vi "CARRITO.vi"() -> ()   [LabVIEW 2021]
uses:
  <vilib>/Instr/_visa.llb/VISA Configure Serial Port (Instr).vi
  <vilib>/Utility/inputDevices.llb/keyboardAcquire.vi
  <vilib>/Utility/inputDevices.llb/closeKeyboard.vi
panel:
  out "servo":dbl(knob) scale=-90.0..90.0
  out "Numeric":dbl
  out "VELOCIDAD":dbl(knob) scale=0.0..100.0
  out "keys pressed":T1(array[ring])
  in  "VISA resource name":refnum<visa-resource-name>
  in  "stop":bool
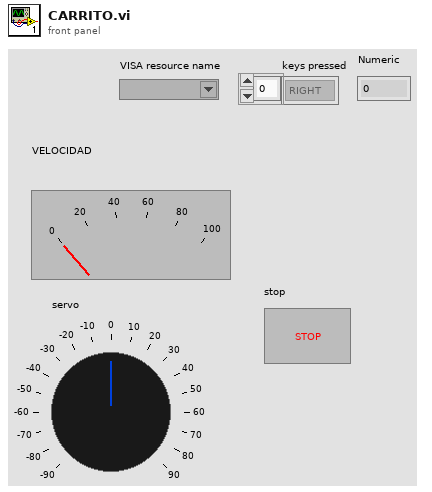
[diagram p1: front panel]
types:
  T1 = enum16{"0", "1", "2", "3", "4", "5", "6", "7", "8", "9", "A", "B", "C", "D", "E", "F", "G", "H", "I", "J", "K", "L", "M", "N", "O", "P", "Q", "R", "S", "T", "U", "V", "W", "X", "Y", "Z", "F1", "F2", "F3", "F4", "F5", "F6", "F7", "F8", "F9", "F10", "F11", "F12", "F13", "F14", "F15", "ADD", "BACK", "BACKSLASH", "CAPITAL", "COMMA", "DECIMAL", "DELETE", "DIVIDE", "DOWN", "END", "EQUALS", "ESCAPE", "GRAVE (`)", "HOME", "INSERT", "LBRACKET", "LCONTROL", "LEFT", "L ALT", "LSHIFT", "LWIN", "MINUS", "MULTIPLY", "NEXT", "NUMLOCK", "NUMPAD_0", "NUMPAD_1", "NUMPAD_2", "NUMPAD_3", "NUMPAD_4", "NUMPAD_5", "NUMPAD_6", "NUMPAD_7", "NUMPAD_8", "NUMPAD_9", "PAUSE", "PERIOD", "PRIOR (PG UP)", "RBRACKET", "RCONTROL", "RETURN", "RIGHT", "R ALT", "RSHIFT", "RWIN", "SCROLL", "SEMICOLON", "SLASH", "SPACE", "SUBTRACT", "TAB", "UP", "ENTER (num pad)", "' (quote)"}[]
  T2 = enum16{"0", "1", "2", "3", "4", "5", "6", "7", "8", "9", "A", "B", "C", "D", "E", "F", "G", "H", "I", "J", "K", "L", "M", "N", "O", "P", "Q", "R", "S", "T", "U", "V", "W", "X", "Y", "Z", "F1", "F2", "F3", "F4", "F5", "F6", "F7", "F8", "F9", "F10", "F11", "F12", "F13", "F14", "F15", "ADD", "BACK", "BACKSLASH", "CAPITAL", "COMMA", "DECIMAL", "DELETE", "DIVIDE", "DOWN", "END", "EQUALS", "ESCAPE", "GRAVE (`)", "HOME", "INSERT", "LBRACKET", "LCONTROL", "LEFT", "L ALT", "LSHIFT", "LWIN", "MINUS", "MULTIPLY", "NEXT", "NUMLOCK", "NUMPAD_0", "NUMPAD_1", "NUMPAD_2", "NUMPAD_3", "NUMPAD_4", "NUMPAD_5", "NUMPAD_6", "NUMPAD_7", "NUMPAD_8", "NUMPAD_9", "PAUSE", "PERIOD", "PRIOR (PG UP)", "RBRACKET", "RCONTROL", "RETURN", "RIGHT", "R ALT", "RSHIFT", "RWIN", "SCROLL", "SEMICOLON", "SLASH", "SPACE", "SUBTRACT", "TAB", "UP", "ENTER (num pad)", "' (quote)"}
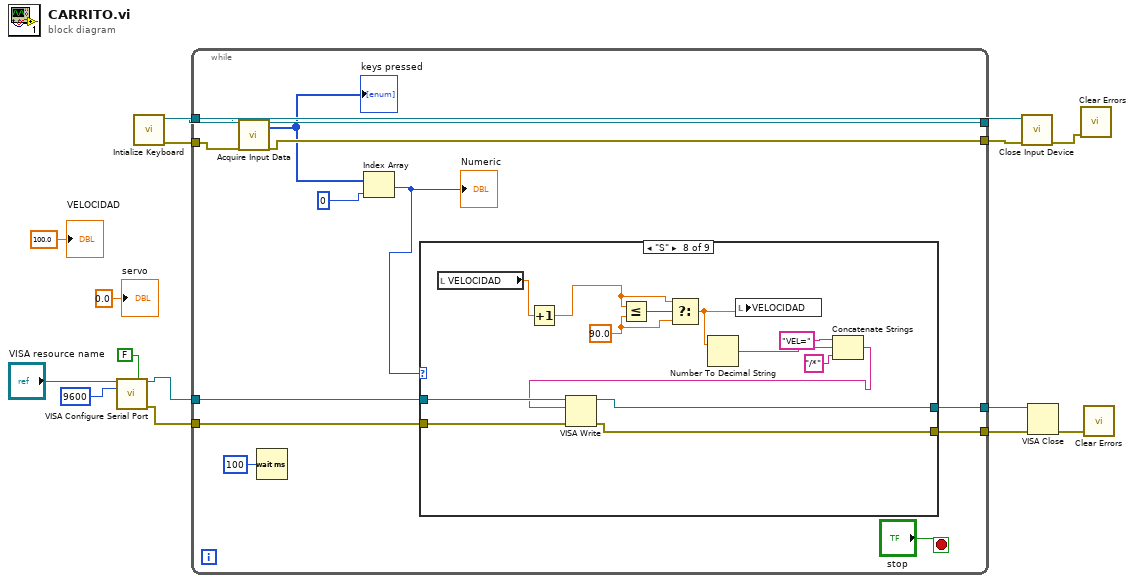
[diagram p0: block diagram]
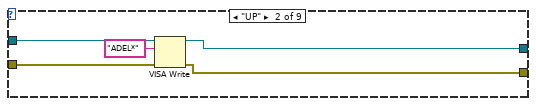
[diagram p3: hidden frame]
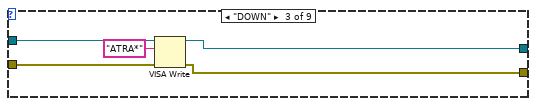
[diagram p4: hidden frame]
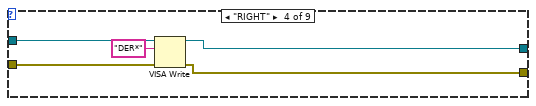
[diagram p5: hidden frame]
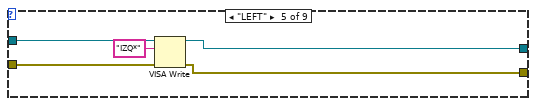
[diagram p6: hidden frame]
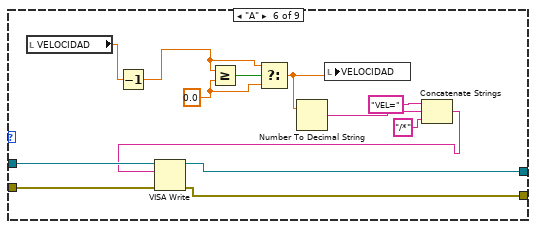
[diagram p7: hidden frame]
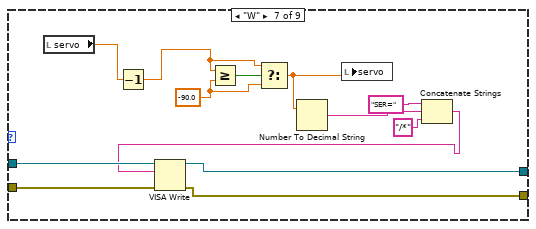
[diagram p8: hidden frame]
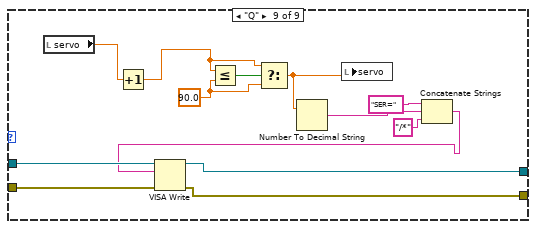
[diagram p9: hidden frame]
diagram:
  n1 = call-poly "VISA Configure Serial Port"("VISA resource name"="VISA resource name", "Enable Termination\nChar (T)"=FALSE ("Enable Termination\nChar (T)"), "baud rate (9600)"=u32 9600) -> ("VISA resource name out"=w8:refnum<visa-resource-name>, "error out"=w7:errorcluster)  [unwired: 11 in]
  n2 = call <vilib>:"Intialize Keyboard.vi"() -> ("error out"=w14:errorcluster, "device ID"=w15:refnum<k1>)  [unwired: 10 in]
  n3 = while {
    tunnel: w15 -> [w28]
    tunnel: w14 -> [w27]
    tunnel: [w26] -> w13
    tunnel: [w25] -> w12
    tunnel: w8 -> [w21]
    tunnel: w7 -> [w20]
    tunnel: [w19] -> w6
    tunnel: [w18] -> w5
    stop <- "stop" stop-if-true
    n4 = call-poly <vilib>:"Acquire Input Data.vi"("device ID"=w28, "error in (no error)"=w27) -> ("device ID"=w26:refnum<k1>, "keys pressed"=w22:T1, "error out"=w25:errorcluster)  [unwired: 15 in]
    "keys pressed" <- w22
    n5 = Wait (ms)(milliseconds to wait=u32 100) -> ()  [unwired: 1 out]
    n6 = Index Array(array=w22, index=0) -> (element=w16:T2)
    "Numeric" <- w16
    n7 = case shown="\"S\"" w16 {
      tunnel: w21 -> [w30 w35 w40 w45 w50 w63 w76 w89 w102]
      tunnel: w20 -> [w29 w34 w39 w44 w49 w62 w75 w88 w101]
      tunnel: [w30 w32 w37 w42 w47 w61 w74 w87 w100] -> w19
      tunnel: [w29 w31 w36 w41 w46 w60 w73 w86 w99] -> w18
      frame "0", Default {
      }
      frame "UP" {
        n8 = VISA Write(VISA resource name=w35, write buffer="ADEL*", error in (no error)=w34) -> (VISA resource name out=w32:refnum<visa-resource-name>, error out=w31:errorcluster)  [unwired: 1 out]
      }
      frame "DOWN" {
        n9 = VISA Write(VISA resource name=w40, write buffer="ATRA*", error in (no error)=w39) -> (VISA resource name out=w37:refnum<visa-resource-name>, error out=w36:errorcluster)  [unwired: 1 out]
      }
      frame "RIGHT" {
        n10 = VISA Write(VISA resource name=w45, write buffer="DER*", error in (no error)=w44) -> (VISA resource name out=w42:refnum<visa-resource-name>, error out=w41:errorcluster)  [unwired: 1 out]
      }
      frame "LEFT" {
        n11 = VISA Write(VISA resource name=w50, write buffer="IZQ*", error in (no error)=w49) -> (VISA resource name out=w47:refnum<visa-resource-name>, error out=w46:errorcluster)  [unwired: 1 out]
      }
      frame "A" {
        w56 = 0.0 ("y")
        n12 = local read "VELOCIDAD"() -> (w59:dbl)
        n13 = Decrement(x=w59) -> (x-1=w57:dbl)
        n14 = Greater Or Equal?(x=w57, y=w56) -> (x >= y?=w58:bool)
        n15 = Select(t=w57, s=w58, f=w56) -> (s? t:f=w54:dbl)
        n16 = Number To Decimal String(number=w54) -> (decimal integer string=w52:string)  [unwired: 1 in]
        n17 = local write "VELOCIDAD"(w54) -> ()
        n18 = Concatenate Strings("VEL=" ("string"), w52, "/*" ("string")) -> (w53:string)
        n19 = VISA Write(VISA resource name=w63, write buffer=w53, error in (no error)=w62) -> (VISA resource name out=w61:refnum<visa-resource-name>, error out=w60:errorcluster)  [unwired: 1 out]
      }
      frame "W" {
        w69 = -90.0 ("y")
        n20 = local read "servo"() -> (w72:dbl)
        n21 = Decrement(x=w72) -> (x-1=w70:dbl)
        n22 = Greater Or Equal?(x=w70, y=w69) -> (x >= y?=w71:bool)
        n23 = Select(t=w70, s=w71, f=w69) -> (s? t:f=w67:dbl)
        n24 = Number To Decimal String(number=w67) -> (decimal integer string=w65:string)  [unwired: 1 in]
        n25 = local write "servo"(w67) -> ()
        n26 = Concatenate Strings("SER=" ("string"), w65, "/*" ("string")) -> (w66:string)
        n27 = VISA Write(VISA resource name=w76, write buffer=w66, error in (no error)=w75) -> (VISA resource name out=w74:refnum<visa-resource-name>, error out=w73:errorcluster)  [unwired: 1 out]
      }
      frame "S" {
        w82 = 90.0 ("y")
        n28 = local read "VELOCIDAD"() -> (w85:dbl)
        n29 = Increment(x=w85) -> (x+1=w83:dbl)
        n30 = Less Or Equal?(x=w83, y=w82) -> (x <= y?=w84:bool)
        n31 = Select(t=w83, s=w84, f=w82) -> (s? t:f=w80:dbl)
        n32 = Number To Decimal String(number=w80) -> (decimal integer string=w78:string)  [unwired: 1 in]
        n33 = local write "VELOCIDAD"(w80) -> ()
        n34 = Concatenate Strings("VEL=" ("string"), w78, "/*" ("string")) -> (w79:string)
        n35 = VISA Write(VISA resource name=w89, write buffer=w79, error in (no error)=w88) -> (VISA resource name out=w87:refnum<visa-resource-name>, error out=w86:errorcluster)  [unwired: 1 out]
      }
      frame "Q" {
        w95 = 90.0 ("y")
        n36 = local read "servo"() -> (w98:dbl)
        n37 = Increment(x=w98) -> (x+1=w96:dbl)
        n38 = Less Or Equal?(x=w96, y=w95) -> (x <= y?=w97:bool)
        n39 = Select(t=w96, s=w97, f=w95) -> (s? t:f=w93:dbl)
        n40 = Number To Decimal String(number=w93) -> (decimal integer string=w91:string)  [unwired: 1 in]
        n41 = local write "servo"(w93) -> ()
        n42 = Concatenate Strings("SER=" ("string"), w91, "/*" ("string")) -> (w92:string)
        n43 = VISA Write(VISA resource name=w102, write buffer=w92, error in (no error)=w101) -> (VISA resource name out=w100:refnum<visa-resource-name>, error out=w99:errorcluster)  [unwired: 1 out]
      }
    }
  }
  n44 = call-poly <vilib>:"Close Input Device.vi"("error in (no error)"=w12, "device ID"=w13) -> ("error out"=w3:errorcluster)  [unwired: 8 in]
  n45 = VISA Close(VISA resource name=w6, error in (no error)=w5) -> (error out=w4:errorcluster)
  n46 = call <vilib>:"Clear Errors.vi"("error in (no error)"=w3) -> ()  [unwired: 5 in, 2 out]
  n47 = call <vilib>:"Clear Errors.vi"("error in (no error)"=w4) -> ()  [unwired: 5 in, 2 out]
  "VELOCIDAD" <- 100.0 ("VELOCIDAD")
  "servo" <- 0.0 ("servo")
